vi "write_String.vi"(8 "错误输入（无错误）":errorcluster, 9 "Value":string, 10 "Address":string, 11 "URL":string="opc://localhost/National Instruments.NIOPCServers.V5/Channel1.Battery_Testing.") -> (0 "error out":errorcluster caption="错误输出", 3 "ok?":bool)   [LabVIEW 2013]
panel:
  out "数据":u16
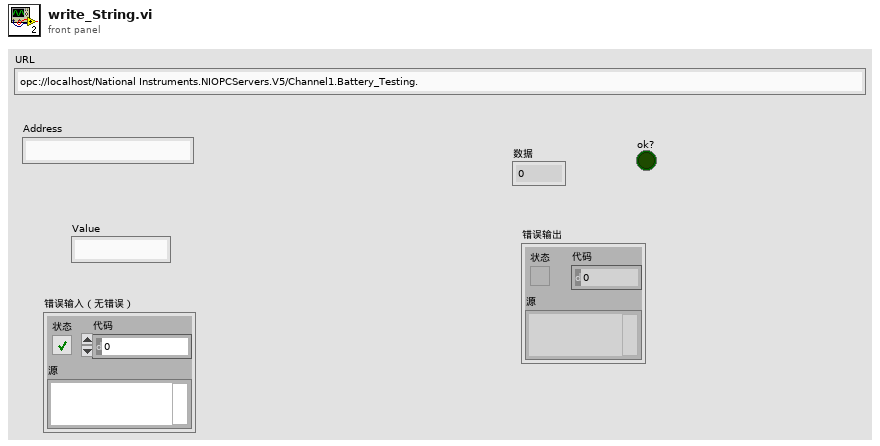
[diagram p1: front panel]
types:
  T1 = enum16{"Read", "Write", "ReadWrite", "BufferedRead", "BufferedReadWrite"}
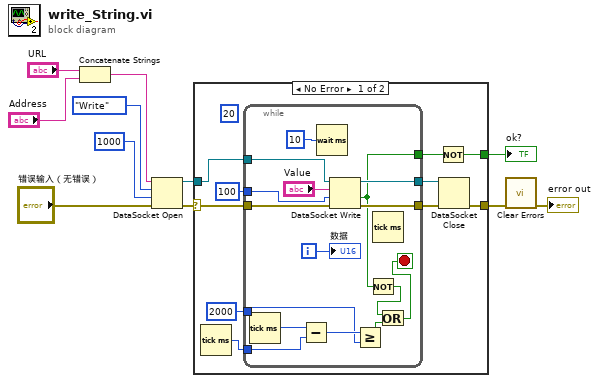
[diagram p0: block diagram]
diagram:
  n1 = Concatenate Strings("URL", "Address") -> (w9:string)
  n2 = DataSocket Open(8:"错误输入（无错误）", 9:1000 ("毫秒超时(10000)"), 10:T1."Write" ("模式"), 11:w9) -> (0:w1:errorcluster, 3:w6:refnum<k13>)
  n3 = case shown="No Error" w1 {
    selector: w1 -> [w14 w38]
    tunnel: w6 -> [w20 _]
    tunnel: [w17 w38] -> w5
    tunnel: [w15 _] -> w3
    frame No Error {
      (unwired) 20
      n4 = Tick Count (ms)() -> (millisecond timer value=w12:u32)
      n5 = while {
        tunnel: 100 ("毫秒超时(0)") -> [w36]
        tunnel: w14 -> [w35]
        tunnel: w20 -> [w34]
        tunnel: [w33] -> w19
        tunnel: [w32] -> w18
        tunnel: [w24] -> w16
        tunnel: 2000 ("毫秒超时(0)") -> [w26]
        tunnel: w12 -> [w25]
        i -> [w30]
        stop <- w22 stop-if-true
        n6 = Tick Count (ms)() -> (millisecond timer value=w27:u32)
        n7 = Subtract(x=w27, y=w25) -> (x-y=w28:u32)
        n8 = Wait (ms)(milliseconds to wait=u32 10 ("等待时间（毫秒）")) -> ()  [unwired: 1 out]
        n9 = DataSocket Write(8:w35, 9:w36, 10:"Value", 11:w34) -> (0:w32:errorcluster, 1:w24:bool, 3:w33:refnum<k13>)
        n10 = Greater Or Equal?(x=w28, y=w26) -> (x >= y?=w29:bool)
        n11 = Not(x=w24) -> (.not. x?=w23:bool)
        n12 = Tick Count (ms)() -> ()  [unwired: 1 out]
        n13 = Or(x=w23, y=w29) -> (x .or. y?=w22:bool)
        "数据" <- w30
      }
      n14 = Not(x=w16) -> (.not. x?=w15:bool)
      n15 = DataSocket Close(8:w18, 11:w19) -> (0:w17:errorcluster)  [unwired: 1 in, 1 out]
    }
    frame Error {
    }
  }
  "ok?" <- w3
  n16 = call <vilib>:"Clear Errors.vi"("error in (no error)"=w5) -> ("error out"=→"error out":errorcluster)  [unwired: 6 in]
